vi "Func - Get argument.vi"(4 "ena NonNum? (F)":bool, 5 "InstanceRef":T1, 6 "error in":bool, 7 "max arg num":i32=100, 8 "arg idx":i32, 9 "arg list":T2[](array[typedef])) -> (0 "error out":bool, 1 "type":u32=1, 2 "str":string, 3 "num":dbl)   [LabVIEW 2021]
doc: "This VI returns the value of the specified function argument. It verifies the total number of actual arguments but does not check argument data types.\n\n<b>arg list</b> specifies the list of function arguments passed to a FuncVI. Wire it to the same terminal on the FuncVI block diagram.\n\n<b>arg idx</b> specifies the index of the desired argument.\n\n<b>max arg num</b> specifies the maximum number of arguments.\n\n<B>ena NonNum</B> enables (TRUE) or disables (FALSE) the ability for the argument to have a data type other than <b>DBL Number</b>.\n\n::: CalcExpress Toolkit :::\nCopyright (c) 2000-2026 Konstantin Shifershteyn. All rights reserved."
uses:
  cetypes.llb/CalcExpress Function Argument Info.ctl
  cetypes.llb/CalcExpress Instance RefNum.ctl
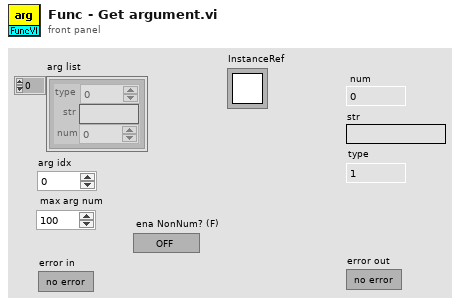
[diagram p1: front panel]
types:
  T1 = typedef "CalcExpress Instance RefNum.ctl" = refnum<k1>
  T2 = typedef "CalcExpress Function Argument Info.ctl" = cluster{"type":u32, "str":string, "num":dbl}
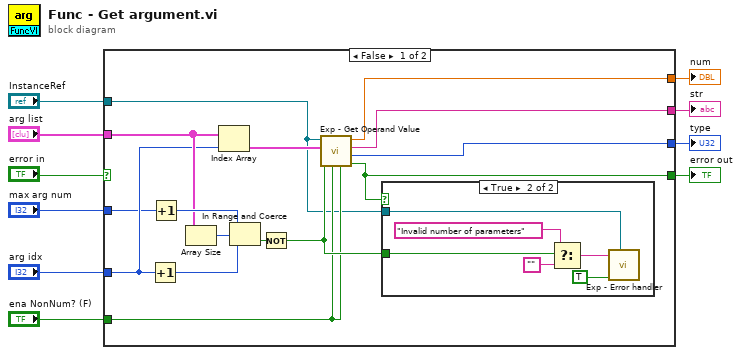
[diagram p0: block diagram]
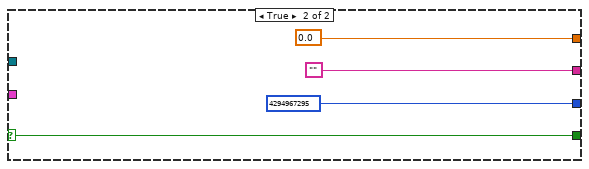
[diagram p3: hidden frame]
diagram:
  n1 = case shown="False" "error in" {
    selector: "error in" -> [_ w32]
    tunnel: [w19 0.0 ("num")] -> w10
    tunnel: [w18 "" ("Empty String Constant")] -> w9
    tunnel: [w17 u32 4294967295 ("type")] -> w8
    tunnel: [w16 w32] -> w7
    tunnel: "arg list" -> [w15 _]
    tunnel: "InstanceRef" -> [w11 _]
    tunnel: "ena NonNum? (F)" -> [w14 _]
    tunnel: "arg idx" -> [w13 _]
    tunnel: "max arg num" -> [w12 _]
    frame False {
      n2 = Increment(x=w13) -> (x+1=w25:i32)
      n3 = Increment(x=w12) -> (x+1=w22:i32)
      n4 = Array Size(array=w15) -> (size(s)=w21:i32)
      n5 = Index Array(array=w15, index=w13) -> (element=w24:T2)
      n6 = In Range and Coerce(upper limit=w22, x=w21, lower limit=w25) -> (In Range?=w20:bool)  [unwired: 1 out]
      n7 = Not(x=w20) -> (.not. x?=w23:bool)
      n8 = call "Exp - Get Operand Value.vi"("ena complex? (F)"=w14, "ena string? (F)"=w14, "error in"=w23, "op info"=w24, "InstanceRef"=w11) -> ("error out"=w16:bool, "type"=w17:u32, "str"=w18:string, "num"=w19:dbl)  [unwired: 1 in]
      n9 = case shown="True" w16 {
        tunnel: w23 -> [_ w31]
        tunnel: w11 -> [_ w26]
        frame False {
        }
        frame True {
          n10 = Select(t="Invalid number of parameters" ("ErrStr"), s=w31, f="" ("Empty String Constant")) -> (s? t:f=w27:string)
          n11 = call "Exp - Error handler.vi"("InstanceRef"=w26, "error in"=TRUE, "error message in"=w27) -> ()  [unwired: 6 in, 3 out]
        }
      }
    }
    frame True {
    }
  }
  "error out" <- w7
  "num" <- w10
  "str" <- w9
  "type" <- w8
